vi "Execute-RT-Benchmarking.vi"   [LabVIEW 2014]
uses:
  <vilib>/Utility/error.llb/DialogType.ctl
  <vilib>/Wiresmith Technology/LabVIEW CLI/CLI Class/CLI.lvclass
types:
  T1 = typedef "DialogType.ctl" = u16
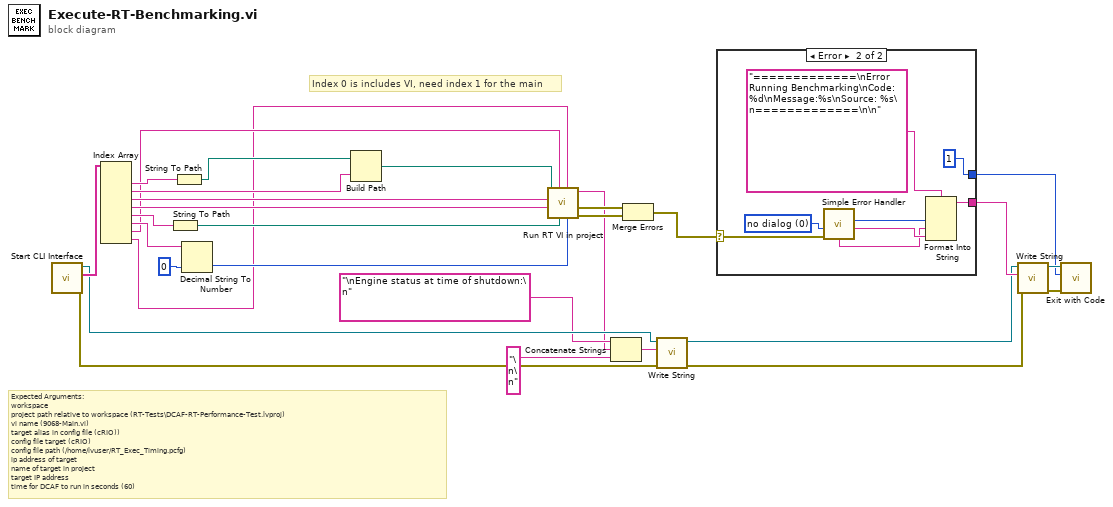
[diagram p0: block diagram]
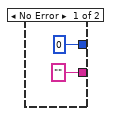
[diagram p2: hidden frame]
diagram:
  # "Index 0 is includes VI, need index 1 for the main"
  # "Expected Arguments:\nworkspace \nproject path relative to workspace (RT-Tests\\DCAF-RT-Performance-Test.lvproj)\nvi name (9068-Main.vi)\ntarget alias in config file (cRIO))\nconfig file target (cRIO)\nconfig file path (/home/lvuser/RT_Exec_Timing.pcfg)\nip address of target\nname of target in project\ntarget IP address\ntime for DCAF to run in seconds (60)"
  n1 = call <vilib>:"Start CLI Interface.vi"() -> ("error out"=w5:errorcluster, "Custom Parameters"=w29:string[], "CLI out"=w8:refnum<class "CLI.lvclass">)  [unwired: 9 in]
  n2 = Index Array(array=w29) -> (element #1=w11:string, element #2=w20:string, element #3=w18:string, element #4=w17:string, element #5=w22:string, element #6=w23:string, element #7=w10:string, element #8=w1:string)  [unwired: 8 in]
  n3 = String To Path(string=w22) -> (path=w16:path)
  n4 = String To Path(string=w11) -> (path=w21:path)
  n5 = Decimal String To Number(string=w23, default (0L)=u32 0 ("default (0 I32)")) -> (number=w15:u32)  [unwired: 1 in, 1 out]
  n6 = Build Path(base path=w21, name or relative path=w20) -> (appended path=w19:path)
  n7 = call "Run RT VI in project.vi"("Run Time"=w15, "project target"=w1, "configuration file path"=w16, "ip address"=w10, "target alias"=w17, "vi name"=w18, "Project Path"=w19) -> ("error out"=w14:errorcluster, "invoked VI error out"=w13:errorcluster, "engine status"=w2:string)  [unwired: 2 in]
  n8 = Concatenate Strings("\nEngine status at time of shutdown:\n" ("string"), w2, "\n\n" ("string")) -> (w9:string)
  n9 = Merge Errors(w13, w14) -> (w12:errorcluster)
  n10 = call <vilib>:"Write String.vi"("error in (no error)"=w5, "Text to Write"=w9, "CLI in"=w8) -> ("error out"=w6:errorcluster, "CLI out"=w7:refnum<class "CLI.lvclass">)  [unwired: 7 in]
  n11 = case shown="Error" w12 {
    selector: w12 -> [_ w36]
    tunnel: ["" w32] -> w26
    tunnel: [0 ("Exit Code (0)") 1 ("Exit Code (0)")] -> w25
    frame No Error {
    }
    frame Error {
      w37 = T1 0 items=["no dialog", "OK message", "continue or stop message", "OK message + warnings", "continue/stop + warnings"] ("type of dialog (OK msg:1)")
      n12 = call <vilib>:"Simple Error Handler.vi"("type of dialog (OK msg:1)"=w37, "error in (no error)"=w36) -> ("code out"=w35:i32, "source out"=w34:string, "message"=w33:string)  [unwired: 3 in, 2 out]
      n13 = Format Into String(format string="=============\nError Running Benchmarking\nCode: %d\nMessage:%s\nSource: %s\n=============\n\n", w35, w33, w34) -> (resulting string=w32:string)  [unwired: 2 in, 1 out]
    }
  }
  n14 = call <vilib>:"Write String.vi"("error in (no error)"=w6, "Text to Write"=w26, "CLI in"=w7) -> ("error out"=w28:errorcluster, "CLI out"=w27:refnum<class "CLI.lvclass">)  [unwired: 7 in]
  n15 = call <vilib>:"Exit with Code.vi"("error in (no error)"=w28, "Exit Code (0)"=w25, "CLI in"=w27) -> ()  [unwired: 8 in, 1 out]
